vi "Tag Expr Test.vi"() -> ()   [LabVIEW 2020]
doc: "_Test_"
uses:
  Tag/Tag.lvclass/Tag.ctl
  Tag Expr/Tag Expr.lvclass
  C:/Program Files (x86)/National Instruments/LabVIEW 2020/vi.lib/LAVA/muParser/mupExpr/mupExpr.lvclass
  Tag Expr/Tag Expr.lvclass/Tag Expr.ctl
  <vilib>/LAVA/muParser/mupExpr/mupExpr.lvclass/mupExpr.ctl
  ca224119-05c6-41cf-9db8-ad80aa452f58.vi
  2f2ee43f-0975-4879-873a-ea0bf2c8b65a.vi
  <vilib>/LAVA/muParser/mupExpr/Eval.vi
  <vilib>/LAVA/muParser/mupExpr/Eval_SglRes.vi
  Tag Expr/Lookup Tag Values.vi
  <vilib>/LAVA/muParser/mupLib/mupEval.vi
  API/Get Tag Value_ByRef.vi
  <vilib>/LAVA/muParser/mupExpr/Set_Var_Value.vi
  <vilib>/LAVA/muParser/mupExpr/Set_MultiVar_Value.vi
  <vilib>/LAVA/muParser/mupLib/mupCheckError.vi
  Tag/Read Value.vi
  Tag/Read Timestamp.vi
  <vilib>/LAVA/muParser/mupExpr/SetVarVal.vi
  <vilib>/LAVA/muParser/mupLib/mupSetVarValue.vi
  Core/Get Delimiter.vi
  <vilib>/Utility/error.llb/Error Cluster From Error Code.vi
  Tag/Set Properties from Initial.vi
  Core/Add Tag.vi
  Tag/Tag.lvclass
panel:
  out "Boolear Result":bool
  out "Result":dbl format="%#_13g"
  in  "Expression":string="50/test2+23+test1"
  out "error out":errorcluster
  out "Variable Names":string[](array[string])
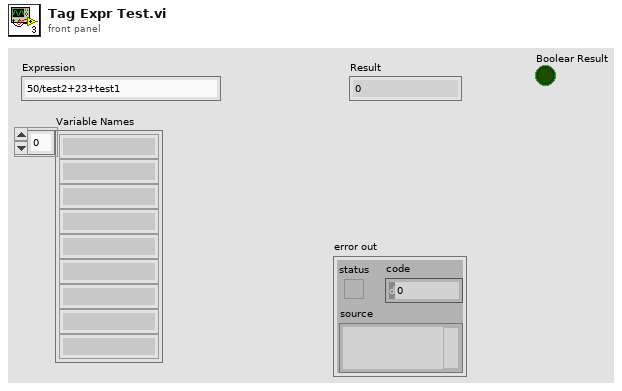
[diagram p1: front panel]
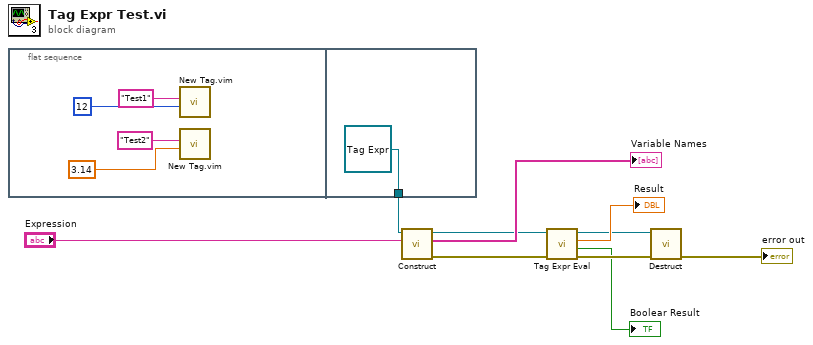
[diagram p0: block diagram]
diagram:
  n1 = flat-sequence {
    tunnel: [refnum<class "Tag Expr.lvclass"> refnum ("CVT Engine:CVT Expr.lvclass")] -> w7
    frame #0 {
      n2 = call "New Tag.vim"("Initial Value"=12, "Tag Name"="Test1" ("Name")) -> ()  [unwired: 8 in, 2 out]
      n3 = call "New Tag.vim"("Initial Value"=3.14, "Tag Name"="Test2" ("Name")) -> ()  [unwired: 8 in, 2 out]
    }
    frame #1 {
    }
  }
  n4 = call-dynamic "Construct.vi"("Expression"="Expression", "Tag Expr in"=w7) -> ("error out"=w5:errorcluster, "Variable Names"=→"Variable Names":string[], "Tag Expr out"=w6:refnum<class "Tag Expr.lvclass">)  [unwired: 6 in, 1 out]
  n5 = call "Tag Expr Eval.vi"("error in (no error)"=w5, "Tag Expr in"=w6) -> ("error out"=w4:errorcluster, "Boolean Result"=→"Boolear Result":bool, "Result"=→"Result":dbl, "Tag Expr out"=w1:refnum<class "Tag Expr.lvclass">)  [unwired: 6 in]
  n6 = call-dynamic "Destruct.vi"("error in (no error)"=w4, "muExpr in"=w1) -> ("error out"=→"error out":errorcluster)  [unwired: 9 in]
